vi "辅助系统全局变量 - T1.vi"() -> ()   [LabVIEW 2026]
panel:
  in  "温度相关数据":T1
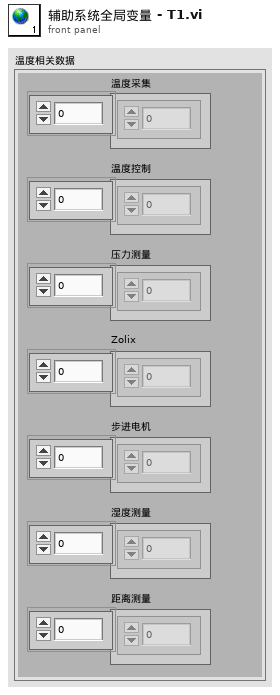
[diagram p1: front panel]
types:
  T1 = typedef "全局变量数据.ctl" = cluster{"温度采集":dbl[], "温度控制":dbl[], "压力测量":dbl[], "Zolix":dbl[], "步进电机":dbl[], "湿度测量":dbl[], "距离测量":dbl[]}
diagram:
